vi "Frame_Get.vi"(8 "error in (no error)":errorcluster, 10 "i":i32, 11 "frames":T2 {"flags" format="%.0x"; "id" format="%.0x"}) -> (0 "error out":errorcluster, 2 "data offset":i32, 3 "frame":T1 {"id" format="%.0x"})   [LabVIEW 2021, in "CANsub_API.lvlib" / "CANsub_Channel.lvclass"]
doc: "Frame i of a CANsub_Frames buffer: id, t_dev, dlc, data len and the 7 flag Booleans (CANsub_Frame), plus data offset = i·64 into frames.data (read the payload there; no copy). i outside 0…count-1 ? 5209. Loop-safe: no allocation, bounded time."
uses:
  CANsub_Channel.lvclass
  Typedefs/CANsub_Frame.ctl
  CANsub_API.lvlib
  Typedefs/CANsub_Frames.ctl
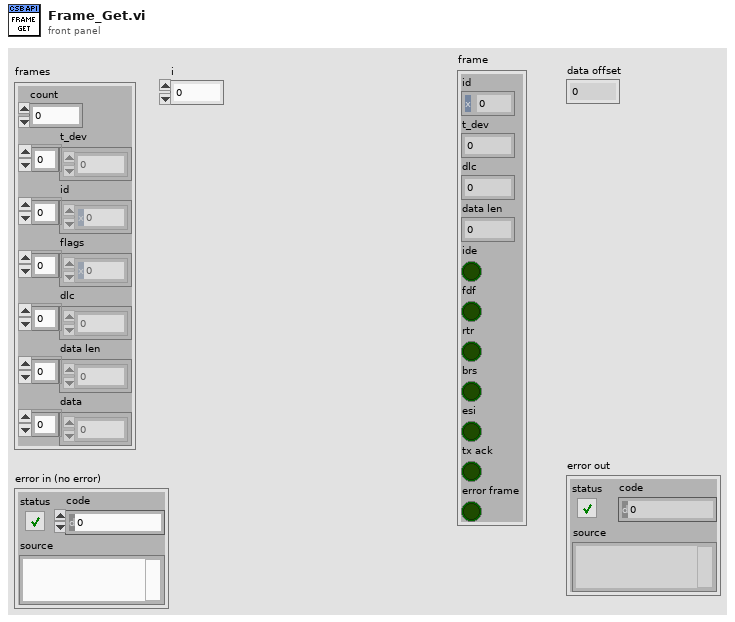
[diagram p1: front panel]
types:
  T1 = typedef "CANsub_API.lvlib/CANsub_Frame.ctl" = cluster{"id":u32, "t_dev":dbl, "dlc":u8, "data len":u8, "ide":bool, "fdf":bool, "rtr":bool, "brs":bool, "esi":bool, "tx ack":bool, "error frame":bool}
  T2 = typedef "CANsub_API.lvlib/CANsub_Frames.ctl" = cluster{"count":i32, "t_dev":dbl[], "id":u32[], "flags":u16[], "dlc":u8[], "data len":u8[], "data":u8[]}
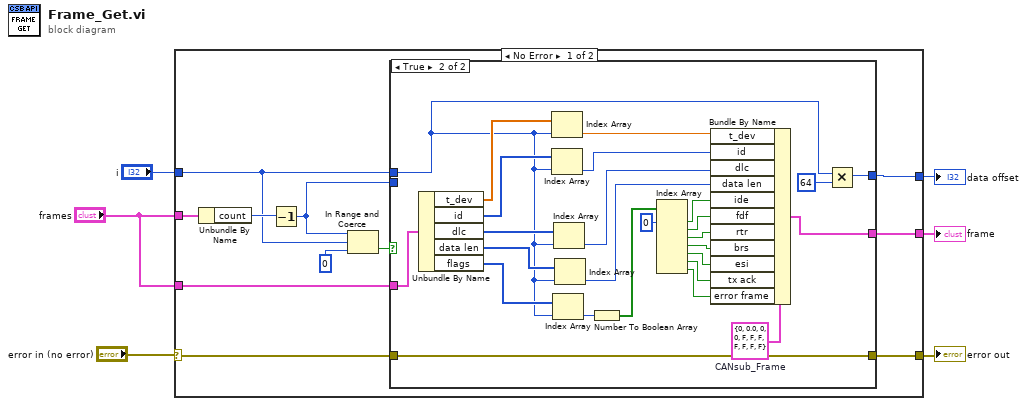
[diagram p0: block diagram]
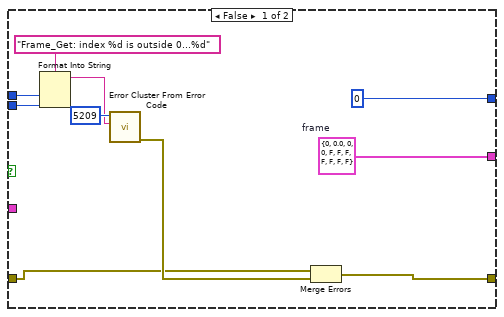
[diagram p2: hidden frame]
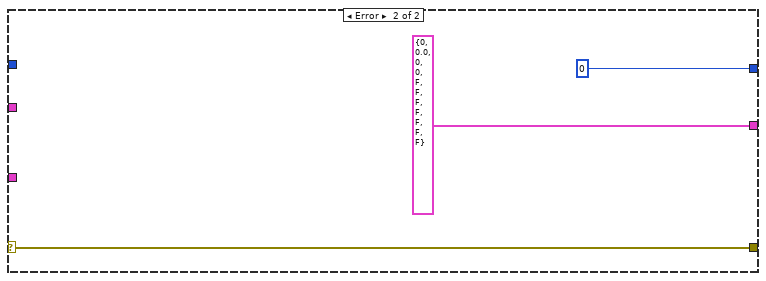
[diagram p3: hidden frame]
diagram:
  n1 = case shown="No Error" "error in (no error)" {
    selector: "error in (no error)" -> [w7 w54]
    tunnel: [w10 0 ("data offset")] -> w5
    tunnel: [w11 T1 {"id"=0, "t_dev"=0.0, "dlc"=0, "data len"=0, "ide"=FALSE, "fdf"=FALSE, "rtr"=FALSE, "brs"=FALSE, "esi"=FALSE, "tx ack"=FALSE, "error frame"=FALSE} ("frame")] -> w4
    tunnel: [w9 w54] -> w3
    tunnel: "frames" -> [w17 _]
    tunnel: "i" -> [w12 _]
    tunnel: "frames" -> [w8 _]
    frame No Error {
      n2 = Unbundle By Name(w17) -> ("count"=w15:i32)
      n3 = Decrement(x=w15) -> (x-1=w13:i32)
      n4 = In Range and Coerce(upper limit=w13, x=w12, lower limit=0) -> (In Range?=w14:bool)  [unwired: 1 out]
      n5 = case shown="True" w14 {
        tunnel: w13 -> [w24 _]
        tunnel: w12 -> [w23 w30]
        tunnel: [w22 w47] -> w11
        tunnel: [0 ("data offset") w31] -> w10
        tunnel: [w19 w28] -> w9
        tunnel: w8 -> [_ w53]
        tunnel: w7 -> [w18 w28]
        frame False {
          w22 = T1 {"id"=0, "t_dev"=0.0, "dlc"=0, "data len"=0, "ide"=FALSE, "fdf"=FALSE, "rtr"=FALSE, "brs"=FALSE, "esi"=FALSE, "tx ack"=FALSE, "error frame"=FALSE}  # frame
          n6 = Format Into String(format string="Frame_Get: index %d is outside 0...%d", w23, w24) -> (resulting string=w26:string)  [unwired: 2 in, 1 out]
          n7 = call <vilib>:"Error Cluster From Error Code.vi"("error message (\"\")"=w26, "error code (0)"=5209) -> ("error out"=w20:errorcluster)  [unwired: 7 in]
          n8 = Merge Errors(w18, w20) -> (w19:errorcluster)
        }
        frame True {
          w48 = T1 {"id"=0, "t_dev"=0.0, "dlc"=0, "data len"=0, "ide"=FALSE, "fdf"=FALSE, "rtr"=FALSE, "brs"=FALSE, "esi"=FALSE, "tx ack"=FALSE, "error frame"=FALSE}  # CANsub_Frame
          n9 = Unbundle By Name(w53) -> ("t_dev"=w52:dbl[], "id"=w51:u32[], "dlc"=w50:u8[], "data len"=w49:u8[], "flags"=w41:u16[])
          n10 = Index Array(array=w52, index=w30) -> (element=w43:dbl)
          n11 = Index Array(array=w51, index=w30) -> (element=w42:u32)
          n12 = Index Array(array=w41, index=w30) -> (element=w46:u16)
          n13 = Index Array(array=w50, index=w30) -> (element=w40:u8)
          n14 = Index Array(array=w49, index=w30) -> (element=w39:u8)
          n15 = Number To Boolean Array(number=w46) -> (Boolean array=w45:bool[])
          n16 = Index Array(array=w45, index #1=0 ("index")) -> (element #1=w38:bool, element #2=w37:bool, element #3=w36:bool, element #4=w35:bool, element #5=w34:bool, element #6=w33:bool, element #7=w32:bool)  [unwired: 6 in]
          n17 = Bundle By Name(cluster=w48, "t_dev"=w43, "id"=w42, "dlc"=w40, "data len"=w39, "ide"=w38, "fdf"=w37, "rtr"=w36, "brs"=w35, "esi"=w34, "tx ack"=w33, "error frame"=w32) -> (w47:T1)
          n18 = Multiply(x=w30, y=64) -> (x*y=w31:i32)
        }
      }
    }
    frame Error {
    }
  }
  "frame" <- w4
  "data offset" <- w5
  "error out" <- w3
